vi "LVDeleteFile_Provider_OnCommand.vi"(10 "Command ID":string, 11 "objects":T1[](array[typedef])) -> ()   [LabVIEW 2020]
uses:
  <resource>/Framework/Providers/API/ItemRef.ctl
panel:
  out "error out":errorcluster
  in  "error in":errorcluster
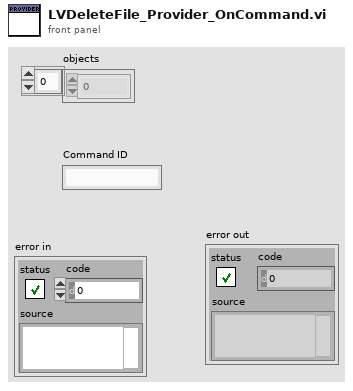
[diagram p1: front panel]
types:
  T1 = typedef "ItemRef.ctl" = u64
  T2 = typedef "ButtonDialogEnum.ctl" = enum16{"Left Button", "Middle Button", "Right Button", "Window Close"}
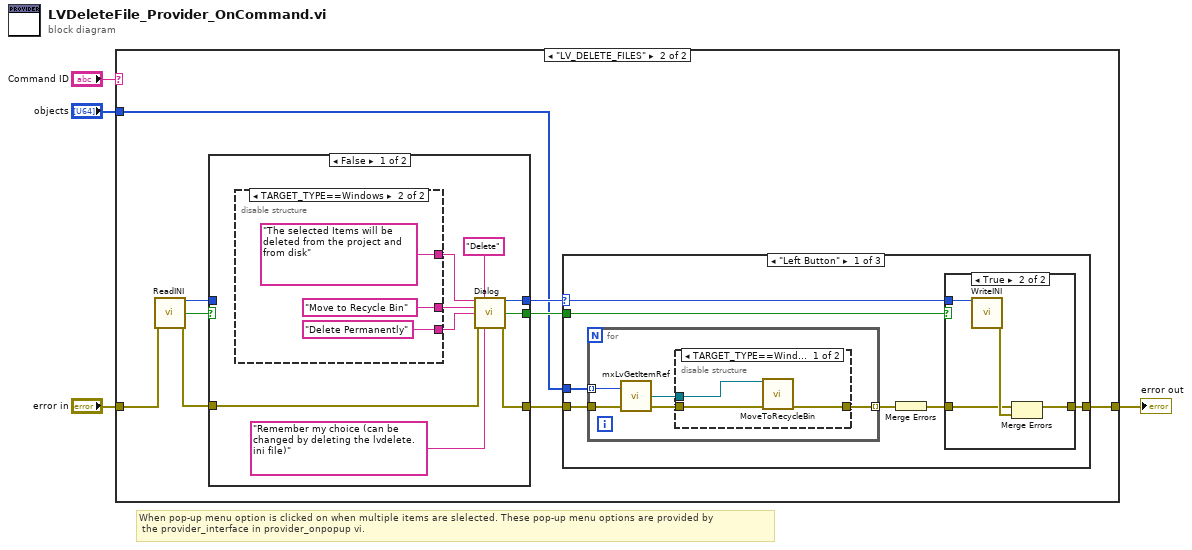
[diagram p0: block diagram]
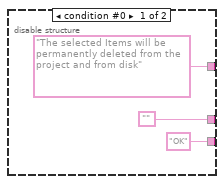
[diagram p3: hidden frame]
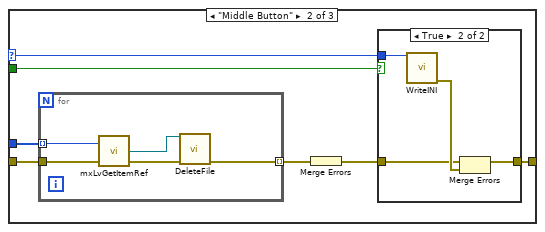
[diagram p7: hidden frame]
diagram:
  # "When pop-up menu option is clicked on when multiple items are slelected. These pop-up menu options are provided by\n the provider_interface in provider_onpopup vi."
  n1 = case shown="\"LV_DELETE_FILES\"" "Command ID" {
    tunnel: "error in" -> [w5 w8]
    tunnel: [w5 w6] -> w1
    tunnel: "objects" -> [_ w7]
    frame Default {
    }
    frame "LV_DELETE_FILES" {
      n2 = call "ReadINI.vi"("error in"=w8) -> ("Button"=w10:T2, "Found?"=w11:bool, "error out"=w12:errorcluster)  [unwired: 12 in]
      n3 = case shown="False" w11 {
        tunnel: [w22 w30] -> w14
        tunnel: [w18 w31] -> w13
        tunnel: w12 -> [w16 w31]
        tunnel: w10 -> [_ w30]
        tunnel: [w15 _] -> w9
        frame False {
          n4 = disable-structure shown="TARGET_TYPE==Windows" {
            disable-tunnel: ["The selected Items will be permanently deleted from the project and from disk" ("message") "The selected Items will be deleted from the project and from disk" ("message")] -> w23
            disable-tunnel: ["" "Move to Recycle Bin" ("message")] -> w21
            disable-tunnel: ["OK" ("message") "Delete Permanently" ("message")] -> w19
            frame condition #0 {
            }
            frame condition #1 (active) {
            }
          }
          n5 = call "Dialog.vi"("Message"=w23, "Title"="Delete" ("Window Title (\"\")"), "LeftButtonText(\"Yes\")"=w21, "MiddleButtonText(\"No\")"=w19, "error in"=w16, "CheckboxText"="Remember my choice (can be changed by deleting the lvdelete.ini file)") -> ("Enum"=w22:T2, "Checked?"=w15:bool, "error out"=w18:errorcluster)  [unwired: 7 in]
        }
        frame True {
        }
      }
      n6 = case shown="\"Left Button\"" w14 {
        selector: w14 -> [w33 w56 _]
        tunnel: w7 -> [w38 w59 _]
        tunnel: w13 -> [w37 w58 w70]
        tunnel: [w35 w54 w70] -> w6
        tunnel: w9 -> [w34 w57 _]
        frame "Left Button" {
          n7 = for {
            tunnel: w38 -> [w43] mode=indexing
            tunnel: w37 -> [w42]
            tunnel: [w39] -> w36 mode=indexing
            n8 = call <resource>:"mxLvGetItemRef.vi"("Item"=w43, "error in"=w42) -> ("Item Refnum"=w41:refnum<vi>, "error out"=w40:errorcluster)  [unwired: 1 out]
            n9 = disable-structure shown="TARGET_TYPE==Windows" {
              disable-tunnel: w41 -> [w46 _]
              disable-tunnel: w40 -> [w45 w47]
              disable-tunnel: [w44 w47] -> w39
              frame condition #0 (active) {
                n10 = call "MoveToRecycleBin.vi"("Item Refnum"=w46, "error in"=w45) -> ("error out"=w44:errorcluster)  [unwired: 13 in]
              }
              frame condition #1 {
              }
            }
          }
          n11 = Merge Errors(w36) -> (w32:errorcluster)
          n12 = case shown="True" w34 {
            tunnel: w32 -> [w48 w49]
            tunnel: [w48 w50] -> w35
            tunnel: w33 -> [_ w51]
            frame False {
            }
            frame True {
              n13 = call "WriteINI.vi"("ButtonEnum"=w51) -> ("error out"=w52:errorcluster)  [unwired: 14 in]
              n14 = Merge Errors(w49, w52) -> (w50:errorcluster)
            }
          }
        }
        frame "Middle Button" {
          n15 = for {
            tunnel: w59 -> [w64] mode=indexing
            tunnel: w58 -> [w63]
            tunnel: [w60] -> w55 mode=indexing
            n16 = call <resource>:"mxLvGetItemRef.vi"("Item"=w64, "error in"=w63) -> ("Item Refnum"=w61:refnum<vi>, "error out"=w62:errorcluster)  [unwired: 1 out]
            n17 = call "DeleteFile.vi"("Item Refnum"=w61, "error in"=w62) -> ("error out"=w60:errorcluster)  [unwired: 13 in]
          }
          n18 = Merge Errors(w55) -> (w53:errorcluster)
          n19 = case shown="True" w57 {
            tunnel: w53 -> [w65 w66]
            tunnel: [w65 w67] -> w54
            tunnel: w56 -> [_ w68]
            frame False {
            }
            frame True {
              n20 = call "WriteINI.vi"("ButtonEnum"=w68) -> ("error out"=w69:errorcluster)  [unwired: 14 in]
              n21 = Merge Errors(w66, w69) -> (w67:errorcluster)
            }
          }
        }
        frame Default {
        }
      }
    }
  }
  "error out" <- w1
